vi "COM test.vi"() -> ()   [LabVIEW 2019]
uses:
  c85feb2e-eb7d-4739-891b-8bfe45c5382b.vi
  0cd483b6-e0b8-416a-96ab-2c8a4a7c8219.vi
  <vilib>/Instr/_visa.llb/VISA Configure Serial Port (Instr).vi
panel:
  out "trimmed string":string
  in  "write buffer":string="M114\n"
  out "return count 2":u32
  out "Serial Settings:Number of Bytes at Serial Port":u32
  out "return count":u32
  out "read buffer":string
  out "error out":errorcluster
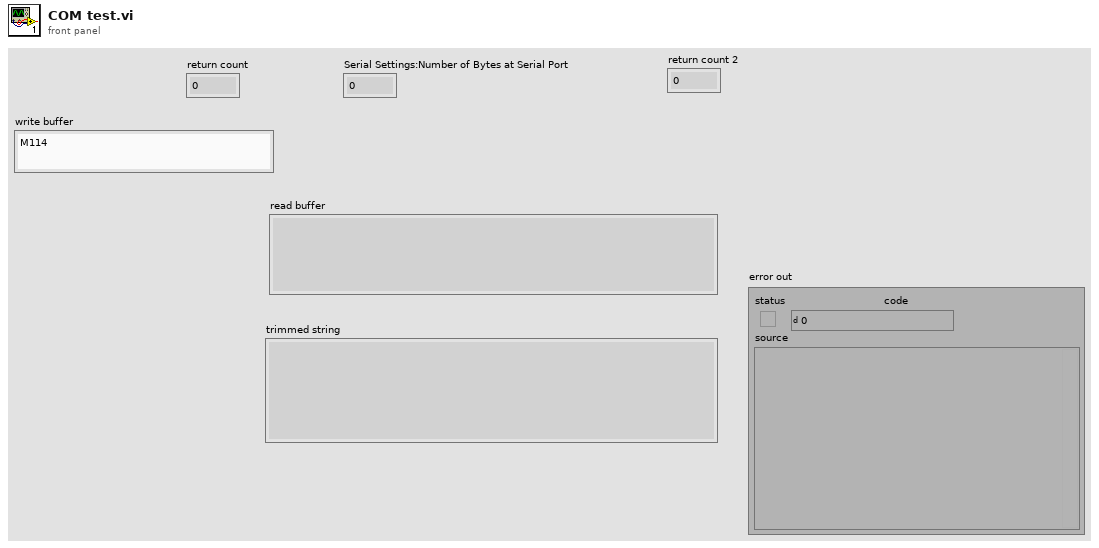
[diagram p1: front panel]
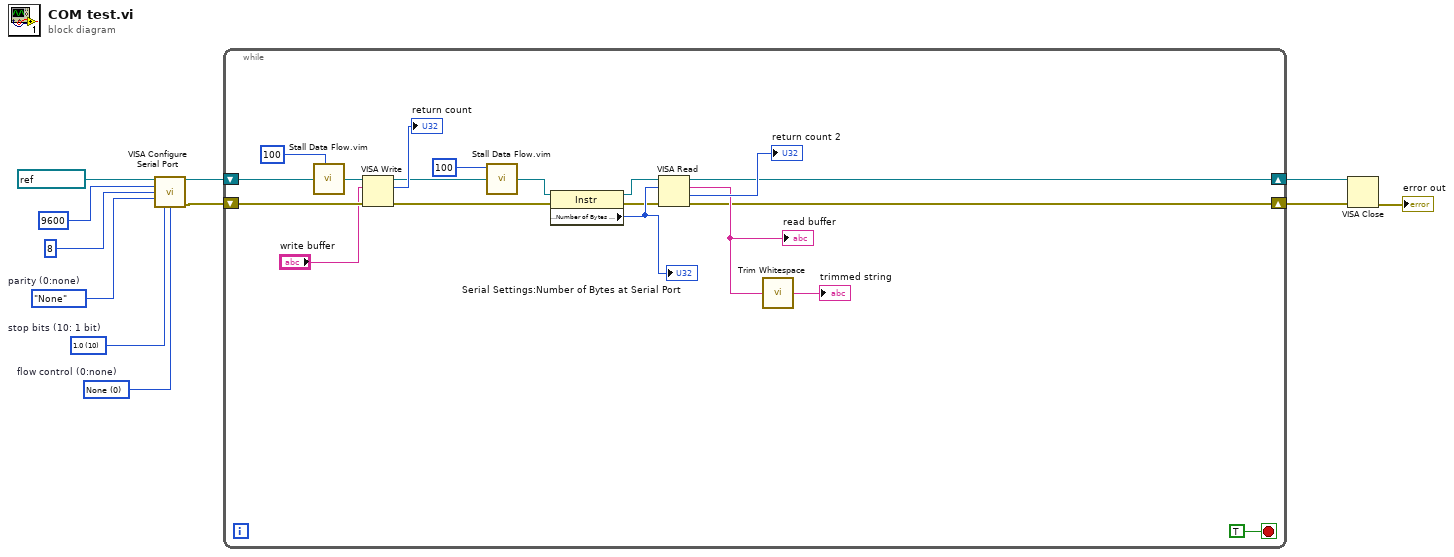
[diagram p0: block diagram]
diagram:
  w1 = u16 0 items=["None", "XON/XOFF", "RTS/CTS", "XON/XOFF & RTS/CTS", "DTR/DSR", "XON/XOFF & DTR/DSR"]  # flow control (0:none)
  w2 = u16 10 items=["1.0"=10, "1.5"=15, "2.0"=20]  # stop bits (10: 1 bit)
  w3 = enum16{"None", "Odd", "Even", "Mark", "Space"}."None"  # parity (0:none)
  n1 = call-poly "VISA Configure Serial Port"("VISA resource name"=refnum<visa-resource-name> "COM21", "baud rate (9600)"=u32 9600, "data bits (8)"=u16 8, "parity (0:none)"=w3, "stop bits (10: 1 bit)"=w2, "flow control (0:none)"=w1) -> ("VISA resource name out"=w8:refnum<visa-resource-name>, "error out"=w7:errorcluster)  [unwired: 8 in]
  n2 = while {
    shift-right: [w18] -> w6
    shift-left: w8 -> [w13]
    shift-right: [w17] -> w5
    shift-left: w7 -> [w26]
    stop <- TRUE stop-if-true
    n3 = call "Stall Data Flow.vim"("value in"=w13, "milliseconds to wait"=u32 100) -> ("value out"=w12:refnum<visa-resource-name>)  [unwired: 1 out]
    n4 = VISA Write(VISA resource name=w12, write buffer="write buffer", error in (no error)=w26) -> (VISA resource name out=w23:refnum<visa-resource-name>, return count=→"return count":u32, error out=w27:errorcluster)
    n5 = call "Stall Data Flow.vim"("value in"=w23, "milliseconds to wait"=u32 100) -> ("value out"=w22:refnum<visa-resource-name>)  [unwired: 1 out]
    n6 = property class="Instr"(reference=w22, error in=w27) -> (reference out=w30:refnum<visa-resource-name>, error out=w28:errorcluster, "Serial Settings:Number of Bytes at Serial Port"=w29:u32)
    "Serial Settings:Number of Bytes at Serial Port" <- w29
    n7 = VISA Read(VISA resource name=w30, byte count=w29, error in (no error)=w28) -> (VISA resource name out=w18:refnum<visa-resource-name>, read buffer=w20:string, return count=→"return count 2":u32, error out=w17:errorcluster)
    "read buffer" <- w20
    n8 = call <vilib>:"Trim Whitespace.vi"("string"=w20) -> ("trimmed string"=→"trimmed string":string)  [unwired: 1 in]
  }
  n9 = VISA Close(VISA resource name=w6, error in (no error)=w5) -> (error out=→"error out":errorcluster)
